vi "KYFG Read Port Reg.vi"(7 "data":u32, 8 "error in (no error)":errorcluster, 9 "address":u64, 10 "port":i32, 11 "handle":u32) -> (0 "error out":errorcluster, 3 "function return":u32(ring), 5 "data out":u32)   [LabVIEW 2023, in "KYFGLib_lv.lvlib"]
doc: "KYFG_API FGSTATUS KYFG_ReadPortReg(FGHANDLE handle, int port, unsigned int address, unsigned int* data);"
uses:
  KYFGLib_lv.lvlib
  KYFGLib.dll
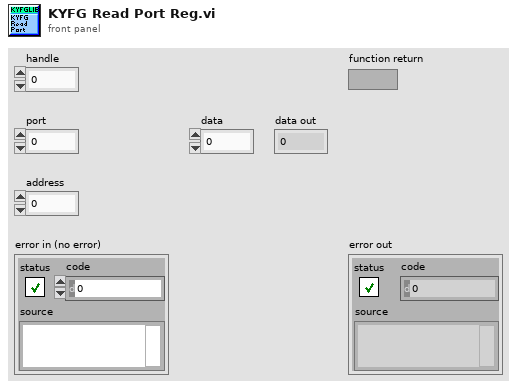
[diagram p1: front panel]
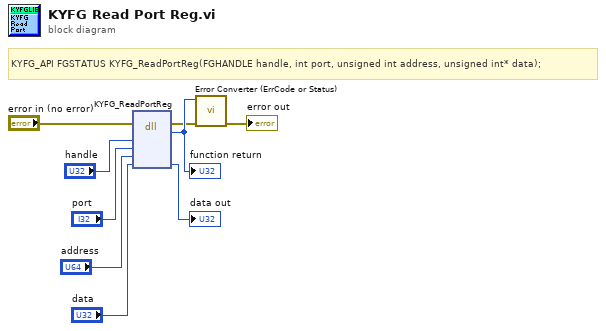
[diagram p0: block diagram]
diagram:
  # "KYFG_API FGSTATUS KYFG_ReadPortReg(FGHANDLE handle, int port, unsigned int address, unsigned int* data);"
  n1 = dll-call lib="KYFGLib.dll" fn="KYFG_ReadPortReg"(error in="error in (no error)", "handle"="handle", "port"="port", "address"="address", "data"="data") -> (error out=w2:errorcluster, "return type"=w9:u32, "data"=→"data out":u32)  [unwired: 5 in, 1 out]
  "function return" <- w9
  n2 = call "Error Converter (ErrCode or Status).vi"("error in (no error)"=w2, "error code"=w9) -> ("error out"=→"error out":errorcluster)  [unwired: 9 in]
